vi "Refresh.vi"(8 "error in (no error)":errorcluster, 11 "Linux System SAL in":refnum<class "Linux System SAL.lvclass">) -> (0 "error out":errorcluster, 3 "Linux System SAL out":refnum<class "Linux System SAL.lvclass">)   [LabVIEW 2020, in "Volatus.lvlib" / "Linux System SAL.lvclass"]
uses:
  Linux System SAL.lvclass
  Linux System SAL.lvclass/Linux System SAL.ctl
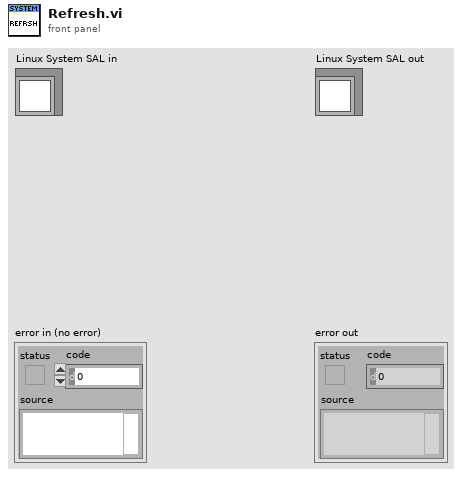
[diagram p1: front panel]
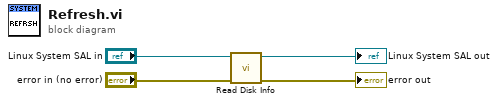
[diagram p0: block diagram]
diagram:
  n1 = call "Read Disk Info.vi"("error in (no error)"="error in (no error)", "Linux System SAL in"="Linux System SAL in") -> ("error out"=→"error out":errorcluster, "Linux System SAL out"=→"Linux System SAL out":refnum<class "Linux System SAL.lvclass">)  [unwired: 8 in]
